vi "RDC-tester.vi"() -> ()   [LabVIEW 2020]
doc: "Test panel, run by hand: builds an element map, calculates the length with RDC-calculate_length and picks specific data points, showing the results on graphs."
uses:
  Reflector/RFH-common_data_format.ctl
  Reflector/RFH-Reflection_File_Handler.lvlib
  RDC-Reflection_Data_Computation.lvlib
panel:
  out "Waveform Graph 2":dbl[](graph)
  out "Waveform Graph":dbl[][](graph)
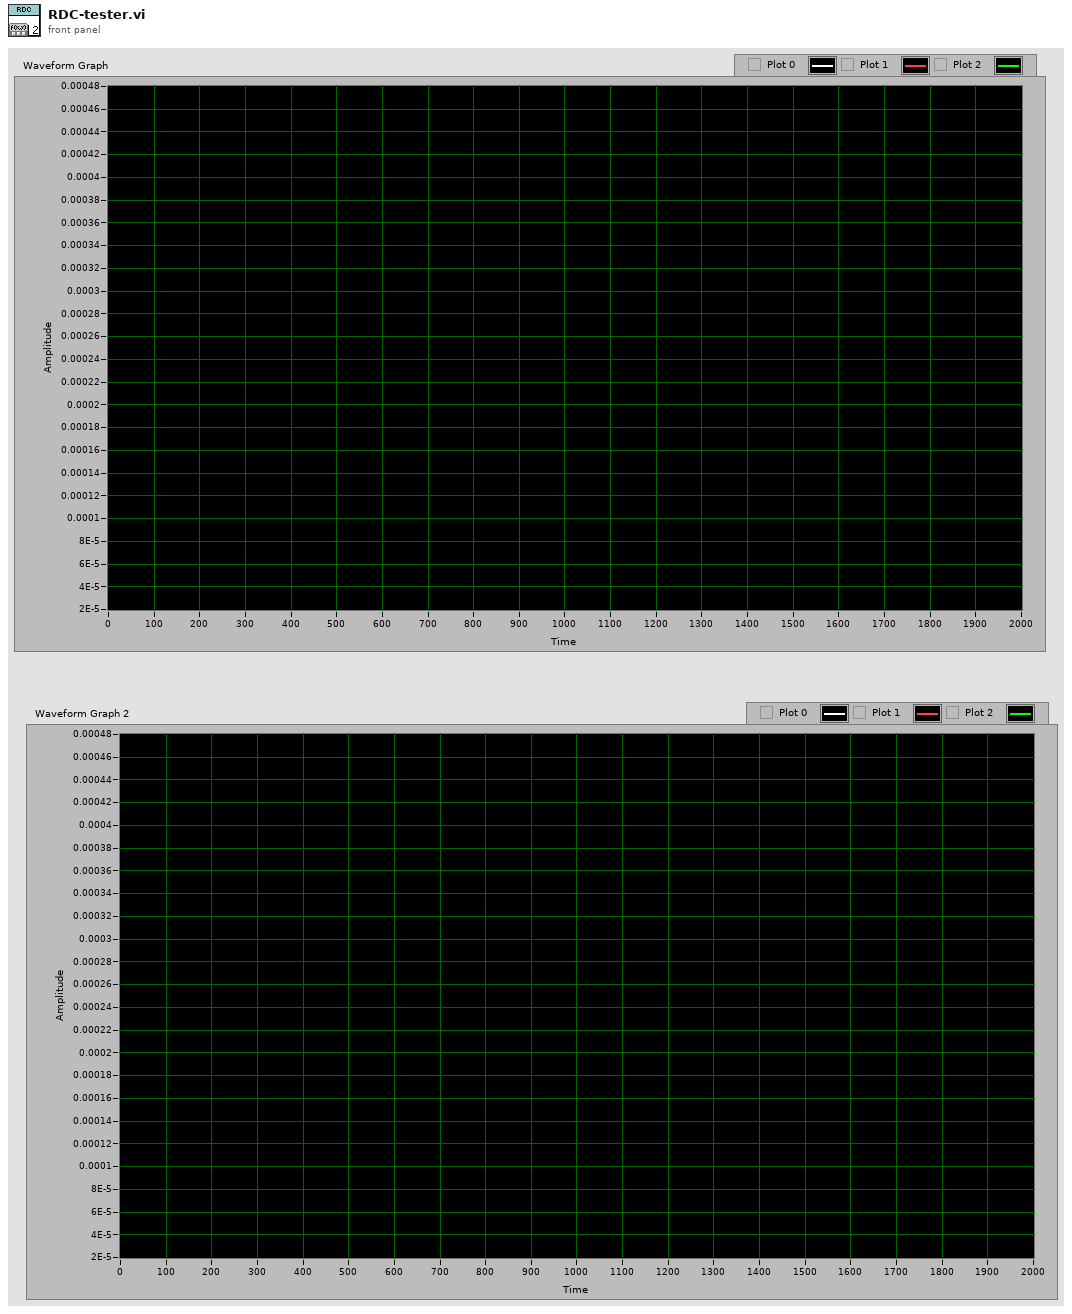
[diagram p1: front panel]
types:
  T1 = typedef "RFH-Reflection_File_Handler.lvlib/RFH-common_data_format.ctl" = cluster{"Frequency":dbl[], "Reflection'":dbl[], "Reflection''":dbl[], "Permativity'":dbl[], "Permativity''":dbl[], "Conductivity":dbl[], "Loss Tangent":dbl[], "Resistance":dbl[], "Reactance":dbl[]}
  T2 = typedef "RFH-Reflection_File_Handler.lvlib/RFH-common_data_format_element.ctl" = cluster{"Frequency":dbl, "Reflection'":dbl, "Reflection''":dbl, "Permativity'":dbl, "Permativity''":dbl, "Conductivity":dbl, "Loss Tangent":dbl, "Resistance":dbl, "Reactance":dbl}
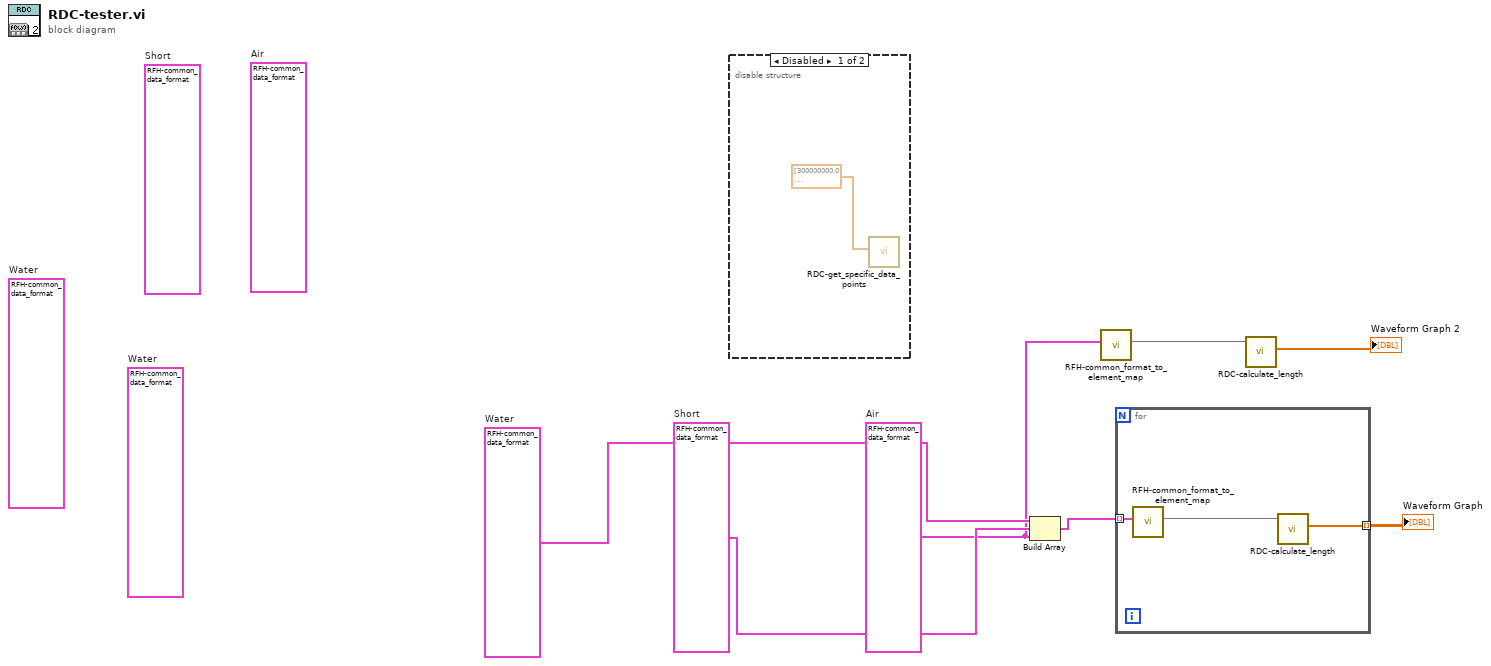
[diagram p0: block diagram]
diagram:
  w7 = T1 {"Frequency"=array[2001 elements], "Reflection'"=array[2001 elements], "Reflection''"=array[2001 elements], "Permativity'"=array[2001 elements], "Permativity''"=array[2001 elements], "Conductivity"=array[2001 elements], "Loss Tangent"=array[2001 elements], "Resistance"=[], "Reactance"=[]}  # Water
  w6 = T1 {"Frequency"=array[2001 elements], "Reflection'"=array[2001 elements], "Reflection''"=array[2001 elements], "Permativity'"=array[2001 elements], "Permativity''"=array[2001 elements], "Conductivity"=array[2001 elements], "Loss Tangent"=array[2001 elements], "Resistance"=[], "Reactance"=[]}  # Short
  w2 = T1 {"Frequency"=array[2001 elements], "Reflection'"=array[2001 elements], "Reflection''"=array[2001 elements], "Permativity'"=array[2001 elements], "Permativity''"=array[2001 elements], "Conductivity"=array[2001 elements], "Loss Tangent"=array[2001 elements], "Resistance"=[], "Reactance"=[]}  # Air
  (unwired) T1 {"Frequency"=array[2001 elements], "Reflection'"=array[2001 elements], "Reflection''"=array[2001 elements], "Permativity'"=array[2001 elements], "Permativity''"=array[2001 elements], "Conductivity"=array[2001 elements], "Loss Tangent"=array[2001 elements], "Resistance"=[], "Reactance"=[]}  # Water
  (unwired) T1 {"Frequency"=array[2001 elements], "Reflection'"=array[2001 elements], "Reflection''"=array[2001 elements], "Permativity'"=array[2001 elements], "Permativity''"=array[2001 elements], "Conductivity"=array[2001 elements], "Loss Tangent"=array[2001 elements], "Resistance"=[], "Reactance"=[]}  # Water
  (unwired) T1 {"Frequency"=array[2001 elements], "Reflection'"=array[2001 elements], "Reflection''"=array[2001 elements], "Permativity'"=array[2001 elements], "Permativity''"=array[2001 elements], "Conductivity"=array[2001 elements], "Loss Tangent"=array[2001 elements], "Resistance"=[], "Reactance"=[]}  # Short
  (unwired) T1 {"Frequency"=array[2001 elements], "Reflection'"=array[2001 elements], "Reflection''"=array[2001 elements], "Permativity'"=array[2001 elements], "Permativity''"=array[2001 elements], "Conductivity"=array[2001 elements], "Loss Tangent"=array[2001 elements], "Resistance"=[], "Reactance"=[]}  # Air
  n1 = disable-structure shown="Disabled" {
    frame Disabled {
      n2 = call "RDC-get_specific_data_points.vi"("Requested Frequencies"=dbl[] [300000000.0, 600000000.0, 1000000000.0, 3000000000.0]) -> ("Element map"=w9:map{dbl, T2})  [unwired: 8 in, 2 out]
    }
    frame Enabled {
    }
  }
  n3 = Build Array(w7, w6, w2) -> (w5:T1[])
  n4 = call "RFH-common_format_to_element_map.vi"("Common Format"=w2) -> ("Element map"=w3:map{dbl, T2})  [unwired: 10 in]
  n5 = for {
    tunnel: w5 -> [w12] mode=indexing
    tunnel: [w10] -> w4 mode=indexing
    n6 = call "RFH-common_format_to_element_map.vi"("Common Format"=w12) -> ("Element map"=w11:map{dbl, T2})  [unwired: 10 in]
    n7 = call "RDC-calculate_length.vi"("Element map"=w11) -> ("L"=w10:dbl[])  [unwired: 10 in]
  }
  "Waveform Graph" <- w4
  n8 = call "RDC-calculate_length.vi"("Element map"=w3) -> ("L"=→"Waveform Graph 2":dbl[])  [unwired: 10 in]
